vi "Host_LogLine.vi"(0 "Surface Defect":string, 1 "Width Defect":string, 2 "Defect":string, 4 "Pitch (mm)":dbl[](array[numeric]), 5 "Width (mm)":dbl, 6 "Dark Pixels":i16, 7 "Result":string, 8 "Pin Count":i32, 9 "Recipe Name":string, 10 "Part ID":u32, 11 "Lot":string) -> (3 "Line":string)   [LabVIEW 2018]
doc: "Use this template to build a VI to use as a subVI."
uses:
  <vilib>/Analysis/NI_AALBase.lvlib
  <vilib>/Analysis/baseanly.llb/Mean (DBL).vi
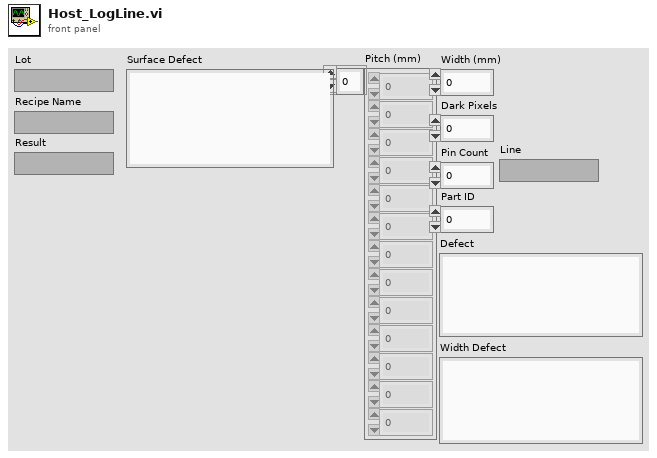
[diagram p1: front panel]
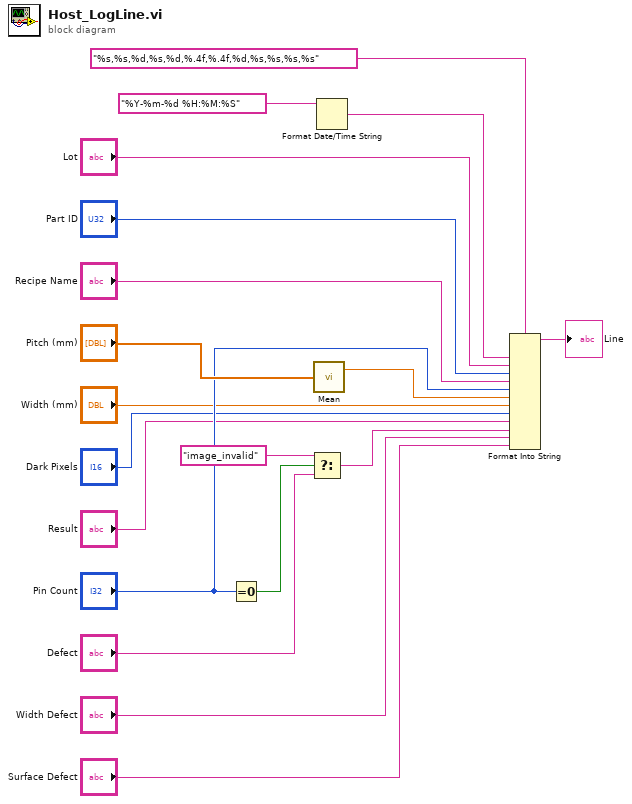
[diagram p0: block diagram]
diagram:
  n1 = Equal To 0?(x="Pin Count") -> (x = 0?=w15:bool)
  n2 = Select(t="image_invalid", s=w15, f="Defect") -> (s? t:f=w4:string)
  n3 = call-poly <vilib>:"Mean.vi"("X"="Pitch (mm)") -> ("mean"=w8:dbl)  [unwired: 1 out]
  n4 = Format Date/Time String(time format string (%c)="%Y-%m-%d %H:%M:%S") -> (date/time string=w12:string)  [unwired: 2 in]
  n5 = Format Into String(format string="%s,%s,%d,%s,%d,%.4f,%.4f,%d,%s,%s,%s,%s", w12, "Lot", "Part ID", "Recipe Name", "Pin Count", w8, "Width (mm)", "Dark Pixels", "Result", w4, "Width Defect", "Surface Defect") -> (resulting string=→"Line":string)  [unwired: 2 in, 1 out]
